vi "Connect.vi"(8 "error in (no error)":errorcluster, 11 "object in":refnum<class "DIO_Channel.lvclass">) -> (0 "error out":errorcluster, 2 "Success?":bool, 3 "object out":refnum<class "DIO_Channel.lvclass">)   [LabVIEW 2021, in "DAQmx.lvlib" / "DIO_Channel.lvclass"]
uses:
  DIO_Channel.lvclass
  C:/Users/averna/Documents/LV Gym DEMO/Factory Pattern/Device Channels/Dependencies/DIO-Channel.lvlibp/Channels/DIO-Channel/DIO_Channel_class/DIO_Channel.lvclass
  DIO_Channel.lvclass/DIO_Channel.ctl
  DIO-Configuration_class/DIO-Configuration.lvclass
  C:/Users/averna/Documents/LV Gym DEMO/Factory Pattern/Device Channels/Dependencies/DIO-Channel.lvlibp/Channels/DIO-Channel/DIO-Configuration_class/DIO-Configuration.lvclass
  Dependencies/DIO-Channel.lvlibp/Channels/DIO-Channel/DIO_Channel_class/Properties/GetDIOConfiguration.vi
  Properties/Get-DIO-DAQmx-Cfg.vi
  <vilib>/DAQmx/create/channels.llb/DAQmx Create Channel (DO-Digital Output).vi
  <vilib>/DAQmx/create/channels.llb/DAQmx Create Channel (DI-Digital Input).vi
  Dependencies/DIO-Channel.lvlibp/Channels/DIO-Channel/DIO-Configuration_class/DIO-Configuration.lvclass
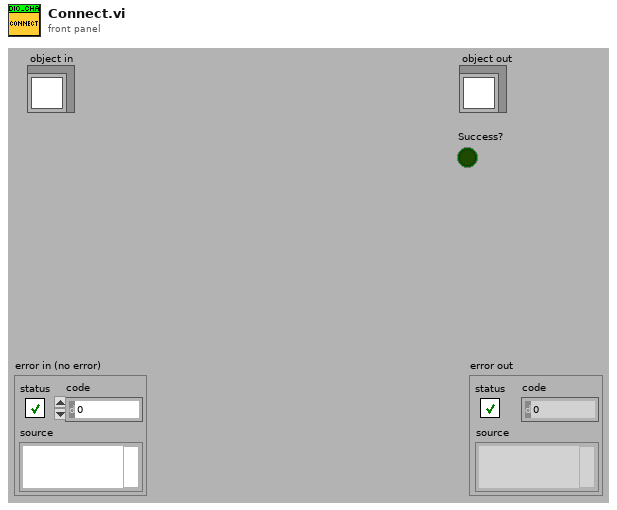
[diagram p1: front panel]
types:
  T1 = typedef "DIO-Channel.lvlibp/DIO-Configuration.lvclass/Direction.ctl" = enum16{"Input", "Output"}
  T2 = typedef "DAQmx.lvlib/DIO-Configuration.lvclass/Data.ctl" = cluster{"DAQ_Line":string}
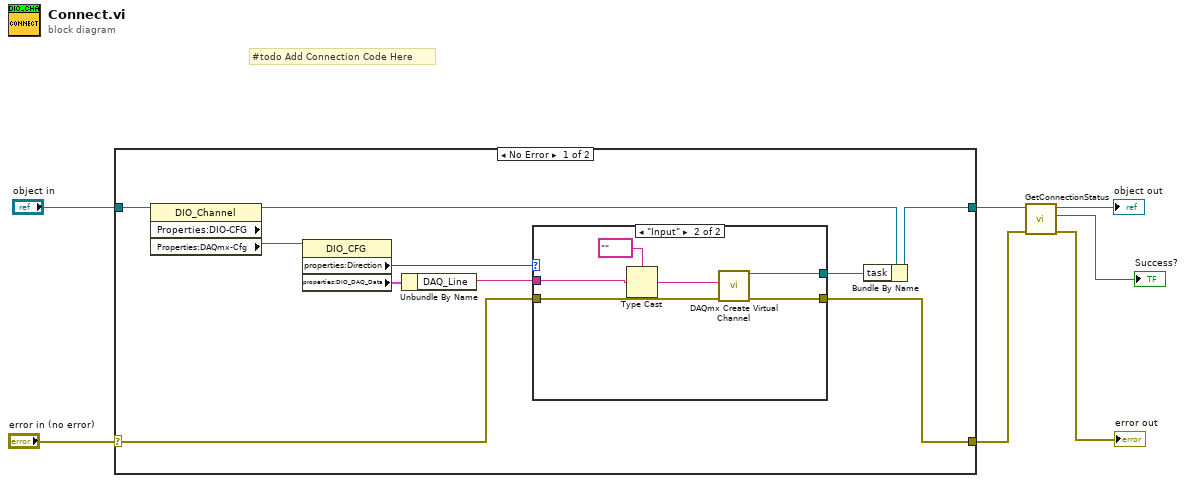
[diagram p0: block diagram]
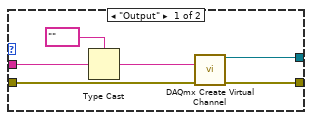
[diagram p2: hidden frame]
diagram:
  # "#todo Add Connection Code Here"
  n1 = case shown="No Error" "error in (no error)" {
    selector: "error in (no error)" -> [w8 w31]
    tunnel: [w9 w31] -> w3
    tunnel: [w16 w30] -> w5
    tunnel: "object in" -> [w17 w30]
    frame No Error {
      n2 = property class="DIO_Channel" props=["Properties:DIO-CFG", "Properties:DAQmx-Cfg"](reference=w17) -> (reference out=w15:refnum<class "DIO_Channel.lvclass">, "Properties:DAQmx-Cfg"=w14:refnum<class "DIO-Configuration.lvclass">)  [unwired: 1 in, 2 out]
      n3 = property class="DIO_CFG"(reference=w14) -> ("properties:Direction"=w12:T1, "properties:DIO_DAQ_Data"=w13:T2)  [unwired: 1 in, 2 out]
      n4 = Unbundle By Name(w13) -> ("DAQ_Line"=w11:string)
      n5 = case shown="\"Input\"" w12 {
        tunnel: w11 -> [w23 w24]
        tunnel: [w22 w29] -> w10
        tunnel: [w20 w28] -> w9
        tunnel: w8 -> [w21 w27]
        frame "Output" {
          n6 = Type Cast(type=tag "" ("lines"), x=w23) -> (*(type *) &x=w18:tag)
          n7 = call-poly <vilib>:"DAQmx Create Virtual Channel.vi"("lines"=w18, "error in"=w21) -> ("task out"=w22:refnum<k21>, "error out"=w20:errorcluster)  [unwired: 12 in]
        }
        frame "Input" {
          n8 = Type Cast(type=tag "" ("lines"), x=w24) -> (*(type *) &x=w25:tag)
          n9 = call-poly <vilib>:"DAQmx Create Virtual Channel.vi"("lines"=w25, "error in"=w27) -> ("task out"=w29:refnum<k21>, "error out"=w28:errorcluster)  [unwired: 12 in]
        }
      }
      n10 = Bundle By Name(cluster=w15, "task"=w10) -> (w16:refnum<class "DIO_Channel.lvclass">)
    }
    frame Error {
    }
  }
  n11 = call-dynamic "GetConnectionStatus.vi"("error in (no error)"=w3, "object in"=w5) -> ("error out"=→"error out":errorcluster, "Connected?"=→"Success?":bool, "object out"=→"object out":refnum<class "DIO_Channel.lvclass">)  [unwired: 7 in]
